vi "Main.vi"() -> ()   [LabVIEW 2025]
uses:
  SubVIs/Arduino_lamps.ctl
  SubVIs/Lamps_global.vi
panel:
  out "EEPROM Erased.":bool
  in  "ESP Port":refnum<visa-resource-name>
  in  "Test Cases":u16(ring) items=["", "Operating Voltage ", "Dynamic InputVoltage", "Over Voltage Test", "Reverse polarity Test", "LUX/ Intensity Test"]
  in  "LAMP COMPONENT":u16(ring) items=["", "HEAD LAMP", "TAIL LAMP", "INDICATORS", "OTHER LAMPS"]
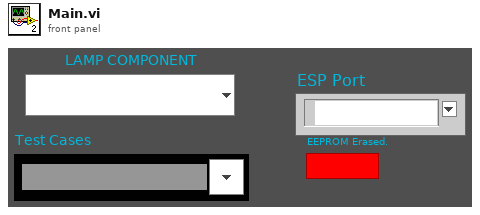
[diagram p1: front panel]
types:
  T1 = typedef "Arduino_lamps.ctl" = enum16{"Init", "Poll", "Read", "Write", "Exit"}
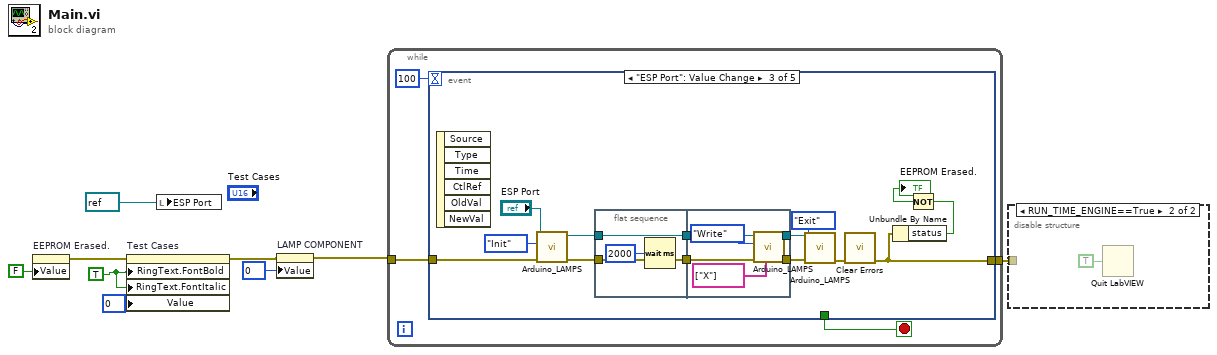
[diagram p0: block diagram]
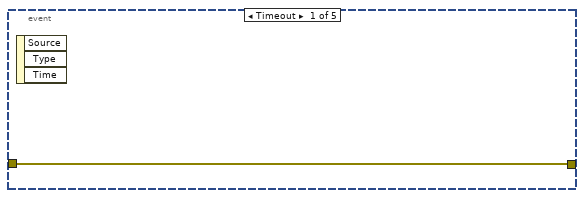
[diagram p3: hidden frame]
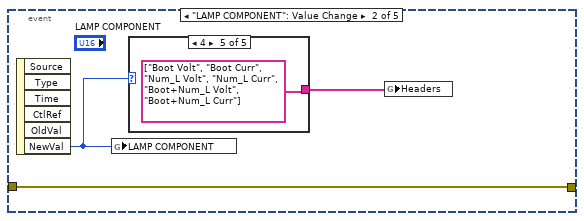
[diagram p4: hidden frame]
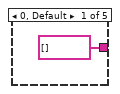
[diagram p5: hidden frame]
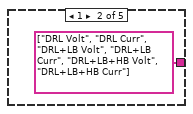
[diagram p6: hidden frame]
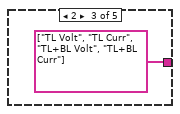
[diagram p7: hidden frame]
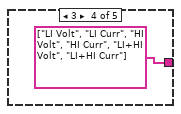
[diagram p8: hidden frame]
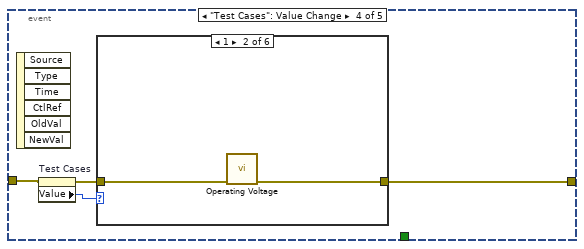
[diagram p9: hidden frame]
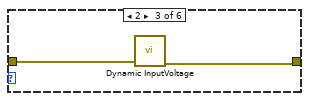
[diagram p11: hidden frame]
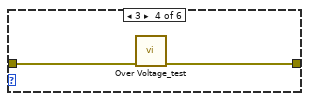
[diagram p12: hidden frame]
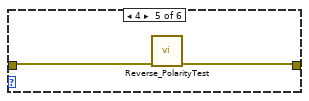
[diagram p13: hidden frame]
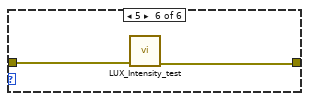
[diagram p14: hidden frame]
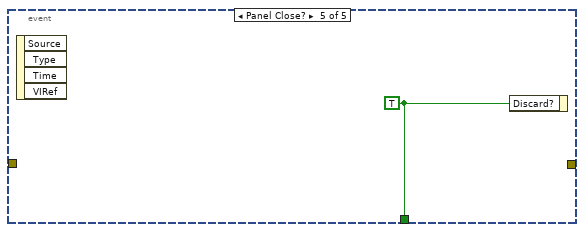
[diagram p15: hidden frame]
diagram:
  w4 = u16 0 items=["", "HEAD LAMP", "TAIL LAMP", "INDICATORS", "OTHER LAMPS"] ("LAMP COMPONENT")
  w7 = u16 0 items=["", "Operating Voltage ", "Dynamic InputVoltage", "Over Voltage Test", "Reverse polarity Test", "LUX/ Intensity Test"] ("Test Cases")
  w8 = TRUE ("Ring Text.Font:Bold")
  n1 = property on="EEPROM Erased." class="Bool (strict)"("Value"=FALSE ("EEPROM Erased.")) -> (error out=w2:errorcluster)  [unwired: 2 in, 1 out]
  n2 = property on="Test Cases" class="Ring (strict)"(error in=w2, "RingText.FontBold"=w8, "RingText.FontItalic"=w8, "Value"=w7) -> (error out=w6:errorcluster)  [unwired: 1 in, 1 out]
  n3 = local write "ESP Port"(refnum<visa-resource-name> refnum ("ESP Port")) -> ()
  n4 = property on="LAMP COMPONENT" class="Ring (strict)"(error in=w6, "Value"=w4) -> (error out=w5:errorcluster)  [unwired: 1 in, 1 out]
  n5 = while {
    tunnel: w5 -> [w11]
    tunnel: [w10] -> w9
    stop <- w12 stop-if-true
    n6 = event shown="[2] \"ESP Port\": Value Change" {
      selector: _ -> [_ _ _ _ _]
      dyn-events: _ -> [_ _ _ _ _]
      timeout: 100 -> [_ _ _ _ _]
      tunnel: [_ _ _ _ w61] -> w12
      tunnel: w11 -> [w14 w17 w35 w48 _]
      tunnel: [w14 w17 w25 w49 _] -> w10
      event Timeout {
        n7 = event-data() -> ()  [unwired: 1 in, 3 out]
      }
      event "LAMP COMPONENT": Value Change {
        n8 = event-data() -> ("NewVal"=w16:u16)  [unwired: 1 in, 5 out]
        n9 = global write "Lamps_global.vi" "LAMP COMPONENT"(w16) -> ()
        n10 = case shown="4" w16 {
          tunnel: [string[] [] string[] ["DRL Volt", "DRL Curr", "DRL+LB Volt", "DRL+LB Curr", "DRL+LB+HB Volt", "DRL+LB+HB Curr"] string[] ["TL Volt", "TL Curr", "TL+BL Volt", "TL+BL Curr"] string[] ["LI Volt", "LI Curr", "HI Volt", "HI Curr", "LI+HI Volt", "LI+HI Curr"] string[] ["Boot Volt", "Boot Curr", "Num_L Volt", "Num_L Curr", "Boot+Num_L Volt", "Boot+Num_L Curr"]] -> w15
          frame 0, Default {
          }
          frame 1 {
          }
          frame 2 {
          }
          frame 3 {
          }
          frame 4 {
          }
        }
        n11 = global write "Lamps_global.vi" "Headers"(w15) -> ()
      }
      event "ESP Port": Value Change {
        n12 = event-data() -> ()  [unwired: 1 in, 6 out]
        n13 = call "Arduino_LAMPS.vi"("error out"=w35, "Enum"=Arduino_lamps."Init", "VISA resource name"="ESP Port") -> ("error out 2"=w32:errorcluster, "VISA out"=w33:refnum<visa-resource-name>)  [unwired: 4 in, 3 out]
        n14 = flat-sequence {
          tunnel: w32 -> [w38]
          tunnel: w33 -> [w39]
          tunnel: [w39] -> w28
          tunnel: [w38] -> w27
          tunnel: [w41] -> w31
          tunnel: [w40] -> w30
          tunnel: w28 -> [w45]
          tunnel: w27 -> [w44]
          frame #0 {
            n15 = Wait (ms)(milliseconds to wait=u32 2000) -> ()  [unwired: 1 out]
          }
          frame #1 {
            n16 = call "Arduino_LAMPS.vi"("DO's"=string[] ["X"], "error out"=w44, "Enum"=Arduino_lamps."Write", "VISA resource name"=w45) -> ("error out 2"=w41:errorcluster, "VISA out"=w40:refnum<visa-resource-name>)  [unwired: 3 in, 3 out]
          }
        }
        n17 = call "Arduino_LAMPS.vi"("error out"=w31, "Enum"=Arduino_lamps."Exit", "VISA resource name"=w30) -> ("error out 2"=w26:errorcluster)  [unwired: 4 in, 4 out]
        n18 = call <vilib>:"Clear Errors.vi"("error in (no error)"=w26) -> ("error out"=w25:errorcluster)  [unwired: 5 in, 1 out]
        n19 = Unbundle By Name(w25) -> ("status"=w24:bool)
        n20 = Not(x=w24) -> (.not. x?=→"EEPROM Erased.":bool)
      }
      event "Test Cases": Value Change {
        n21 = event-data() -> ()  [unwired: 1 in, 6 out]
        n22 = property on="Test Cases" class="Ring (strict)"(error in=w48) -> (error out=w47:errorcluster, "Value"=w46:u16)  [unwired: 1 in, 1 out]
        n23 = case shown="1" w46 {
          tunnel: w47 -> [w50 w52 w54 w56 w58 w60]
          tunnel: [w50 w51 w53 w55 w57 w59] -> w49
          frame 0, Default {
          }
          frame 1 {
            n24 = call "Operating Voltage.vi"("error in (no error)"=w52) -> ("error out"=w51:errorcluster)  [unwired: 10 in]
          }
          frame 2 {
            n25 = call "Dynamic InputVoltage.vi"("error in (no error)"=w54) -> ("error out"=w53:errorcluster)  [unwired: 10 in]
          }
          frame 3 {
            n26 = call "Over Voltage_test.vi"("error in (no error)"=w56) -> ("error out"=w55:errorcluster)  [unwired: 10 in]
          }
          frame 4 {
            n27 = call "Reverse_PolarityTest.vi"("error in (no error)"=w58) -> ("error out"=w57:errorcluster)  [unwired: 10 in]
          }
          frame 5 {
            n28 = call "LUX_Intensity_test.vi"("error in (no error)"=w60) -> ("error out"=w59:errorcluster)  [unwired: 10 in]
          }
        }
      }
      event Panel Close? {
        w61 = TRUE ("Discard?")
        n29 = event-data() -> ()  [unwired: 1 in, 4 out]
        n30 = event-data("Discard?"=w61) -> ()  [unwired: 1 in, 1 out]
      }
    }
  }
  n31 = disable-structure shown="RUN_TIME_ENGINE==True" {
    disable-tunnel: w9 -> [_ _]
    frame condition #0 (active) {
    }
    frame condition #1 {
      n32 = Quit LabVIEW(quit? (T)=TRUE) -> ()
    }
  }
